vi "ASD Right Sequence Formation.vi"(11 "Sample Sequence":string="TGTXCT") -> (0 "RRS#":i32, 3 "RR Seq":T1)   [LabVIEW 2018]
panel:
  out "逆前削減配列マトリクス":string[][](array[string])
  out "順前削減配列マトリクス":string[][](array[string])
  out "Base#":i32[](array[numeric])
  out "Direction":enum16{"5’→3'", "3'→5'"}[](array[ring])
  out "サイズ":i32
  out "Sequence":string[](array[string])
  out "出力クラスタ":T1
  out "付加配列":string[](array[string])
  out "5' to 3'":string[](array[string])
  out "3' to 5'":string[](array[string])
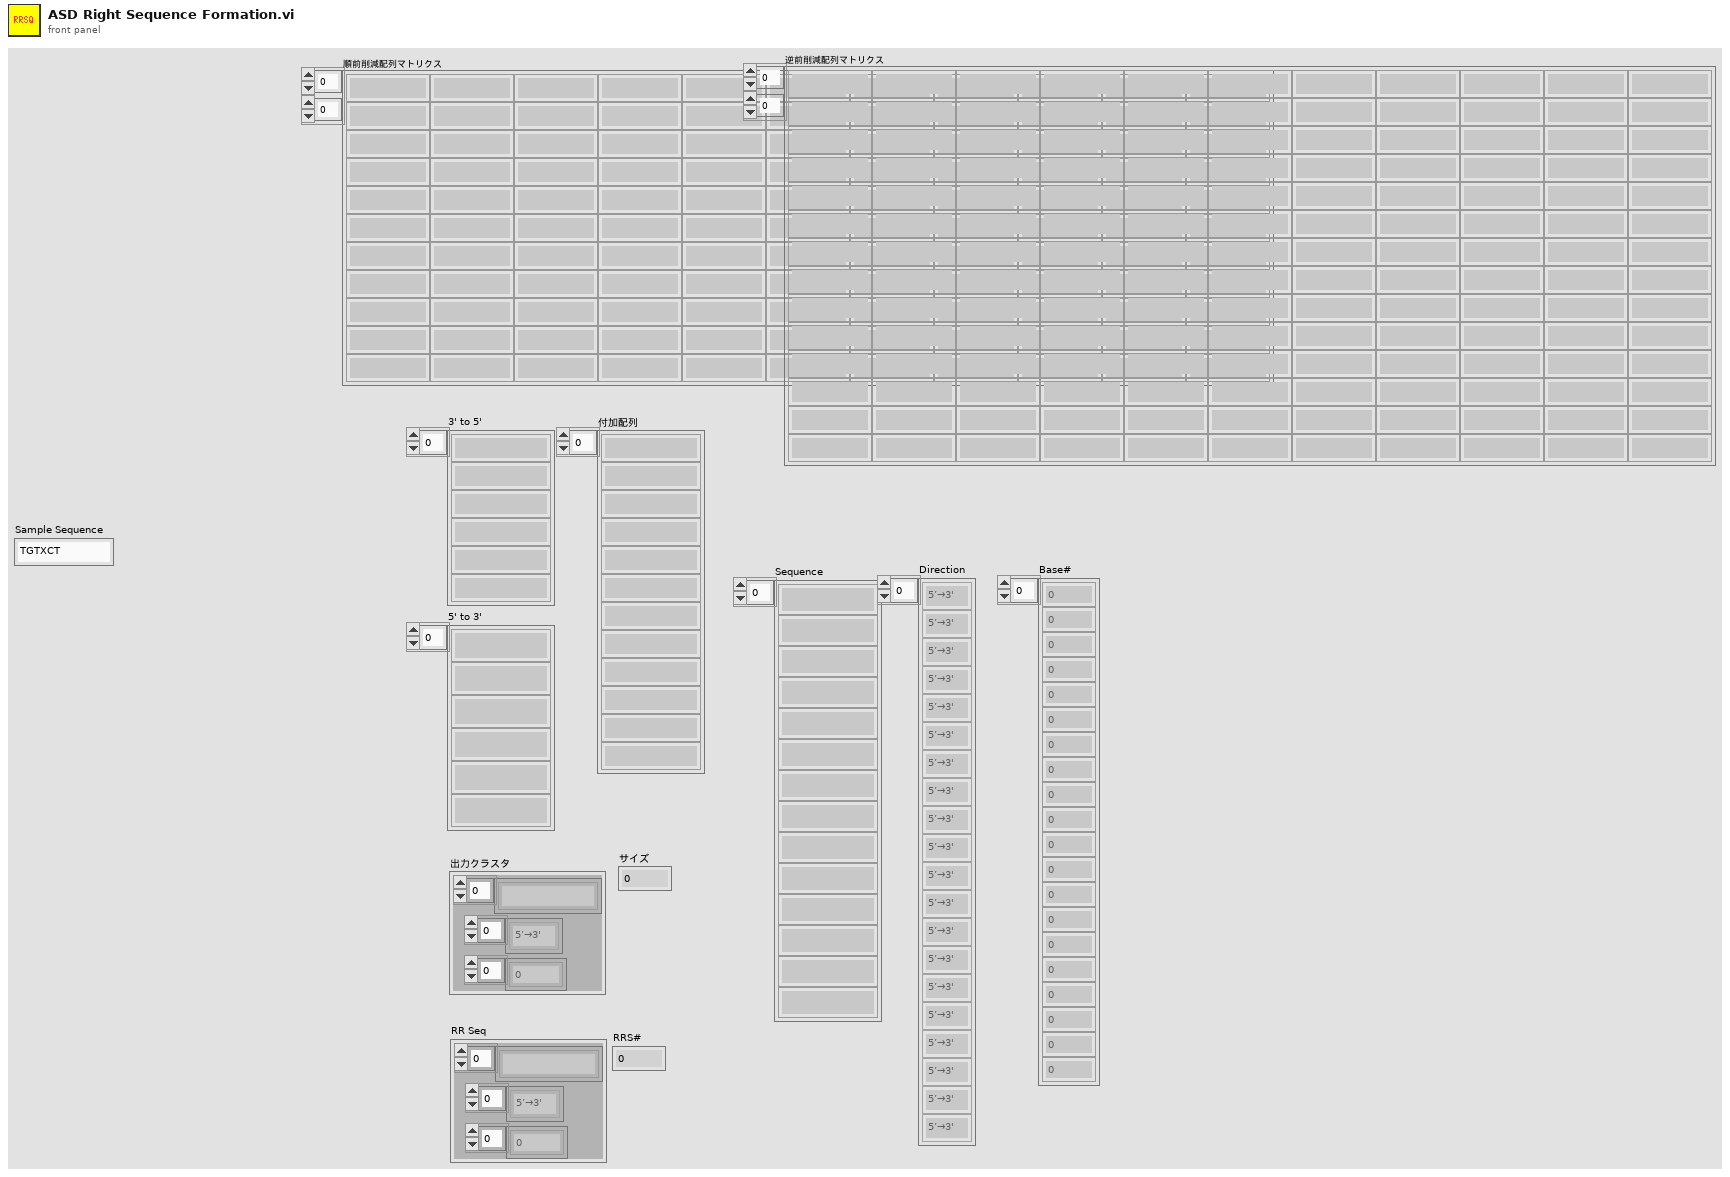
[diagram p1: front panel]
types:
  T1 = cluster{string[], enum16{"5’→3'", "3'→5'"}[], i32[]}
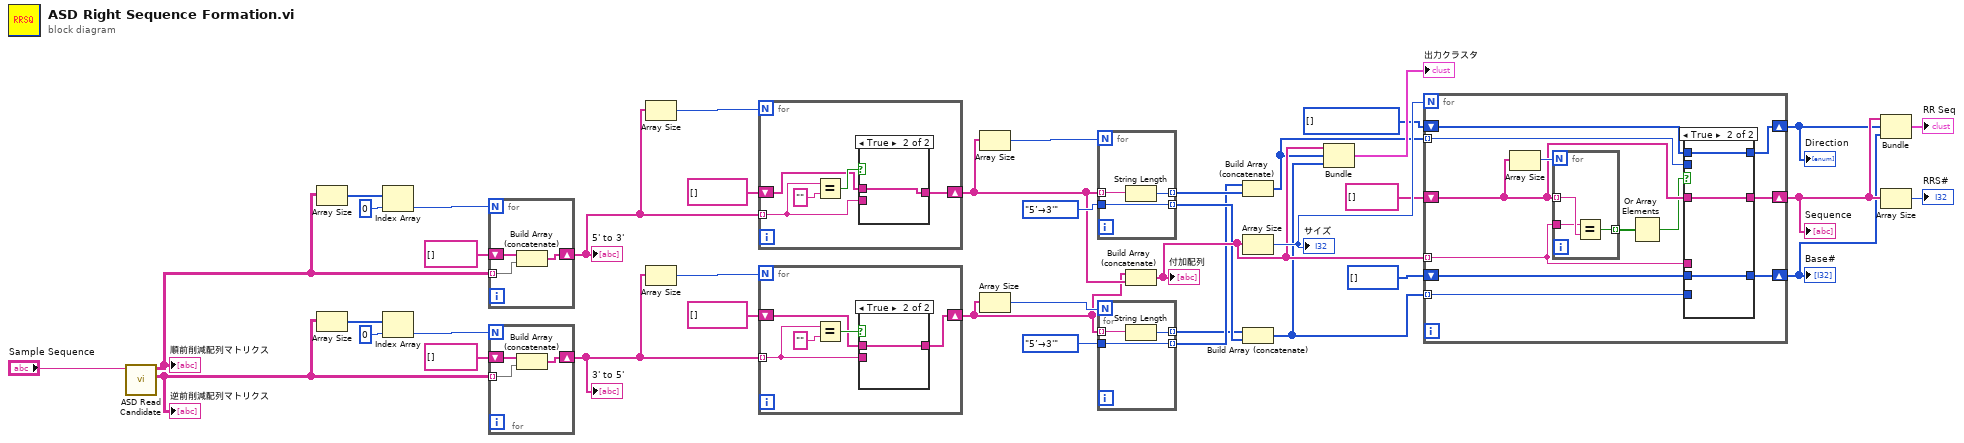
[diagram p0: block diagram]
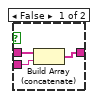
[diagram p2: hidden frame]
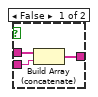
[diagram p3: hidden frame]
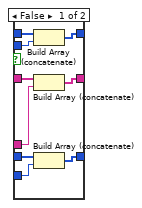
[diagram p4: hidden frame]
diagram:
  w33 = enum16{"5’→3'", "3'→5'"}[] [] items=["5’→3'", "3'→5'"]
  n1 = call "ASD Read Candidate.vi"("読み取り配列"="Sample Sequence") -> ("逆前削減配列マトリクス"=w15:string[][], "順前削減配列マトリクス"=w24:string[][])  [unwired: 8 in, 1 out]
  "順前削減配列マトリクス" <- w24
  "逆前削減配列マトリクス" <- w15
  n2 = Array Size(array=w24) -> (size(s)=w26:i32[])
  n3 = Array Size(array=w15) -> (size(s)=w19:i32[])
  n4 = Index Array(array=w26, index=0 ("指標")) -> (element=w23:i32)
  n5 = Index Array(array=w19, index=0 ("指標")) -> (element=w17:i32)
  n6 = for {
    N: w23 -> [_]
    tunnel: w24 -> [w43] mode=indexing
    shift-right: [w41] -> w4
    shift-left: string[] [] -> [w42]
    n7 = Build Array (concatenate)(w42, w43) -> (w41:string[])
  }
  "5' to 3'" <- w4
  n8 = for {
    N: w17 -> [_]
    tunnel: w15 -> [w46] mode=indexing
    shift-right: [w44] -> w2
    shift-left: string[] [] -> [w45]
    n9 = Build Array (concatenate)(w45, w46) -> (w44:string[])
  }
  "3' to 5'" <- w2
  n10 = Array Size(array=w4) -> (size(s)=w8:i32)
  n11 = Array Size(array=w2) -> (size(s)=w6:i32)
  n12 = for {
    N: w8 -> [_]
    tunnel: w4 -> [w47] mode=indexing
    shift-right: [w48] -> w3
    shift-left: string[] [] -> [w49]
    n13 = Equal?(x=w47, y="") -> (x = y?=w50:bool)
    n14 = case shown="True" w50 {
      tunnel: w49 -> [w54 w55]
      tunnel: [w53 w55] -> w48
      tunnel: w47 -> [w52 _]
      frame False {
        n15 = Build Array (concatenate)(w54, w52) -> (w53:string[])
      }
      frame True {
      }
    }
  }
  n16 = for {
    N: w6 -> [_]
    tunnel: w2 -> [w56] mode=indexing
    shift-right: [w57] -> w1
    shift-left: string[] [] -> [w58]
    n17 = Equal?(x=w56, y="") -> (x = y?=w59:bool)
    n18 = case shown="True" w59 {
      tunnel: w58 -> [w63 w64]
      tunnel: [w62 w64] -> w57
      tunnel: w56 -> [w61 _]
      frame False {
        n19 = Build Array (concatenate)(w63, w61) -> (w62:string[])
      }
      frame True {
      }
    }
  }
  n20 = Array Size(array=w3) -> (size(s)=w21:i32)
  n21 = Array Size(array=w1) -> (size(s)=w14:i32)
  n22 = for {
    N: w21 -> [_]
    tunnel: enum16{"5’→3'", "3'→5'"}."5’→3'" ("リード方向総合") -> [w67]
    tunnel: [w67] -> w12 mode=indexing
    tunnel: w3 -> [w66] mode=indexing
    tunnel: [w65] -> w11 mode=indexing
    n23 = String Length(string=w66) -> (length=w65:i32)
  }
  n24 = for {
    N: w14 -> [_]
    tunnel: enum16{"5’→3'", "3'→5'"}."5’→3'" ("リード方向総合") -> [w70]
    tunnel: [w70] -> w10 mode=indexing
    tunnel: w1 -> [w69] mode=indexing
    tunnel: [w68] -> w9 mode=indexing
    n25 = String Length(string=w69) -> (length=w68:i32)
  }
  n26 = Build Array (concatenate)(w1, w3) -> (w38:string[])
  "付加配列" <- w38
  n27 = Build Array (concatenate)(w10, w11) -> (w34:i32[])
  n28 = Array Size(array=w38) -> (size(s)=w40:i32)
  "サイズ" <- w40
  n29 = Build Array (concatenate)(w9, w12) -> (w35:i32[])
  n30 = Bundle(w38, w34, w35) -> (→"出力クラスタ":cluster{string[], i32[], i32[]})  [unwired: 1 in]
  n31 = for {
    N: w40 -> [_]
    tunnel: w38 -> [w79] mode=indexing
    shift-right: [w82] -> w31
    shift-left: string[] [] -> [w80]
    tunnel: w35 -> [w73] mode=indexing
    tunnel: w34 -> [w76] mode=indexing
    shift-right: [w75] -> w30
    shift-left: w33 -> [w74]
    shift-right: [w72] -> w29
    shift-left: i32[] [] -> [w71]
    n32 = Array Size(array=w80) -> (size(s)=w81:i32)
    n33 = for {
      N: w81 -> [_]
      tunnel: w80 -> [w97] mode=indexing
      tunnel: w79 -> [w96]
      tunnel: [w95] -> w78 mode=indexing
      n34 = Equal?(x=w96, y=w97) -> (x = y?=w95:bool)
    }
    n35 = Or Array Elements(Boolean array=w78) -> (logical OR=w77:bool)
    n36 = case shown="True" w77 {
      tunnel: [w91 w94] -> w82
      tunnel: w80 -> [w90 w94]
      tunnel: w79 -> [w89 _]
      tunnel: w76 -> [w88 _]
      tunnel: [w87 w93] -> w75
      tunnel: w74 -> [w86 w93]
      tunnel: w73 -> [w85 _]
      tunnel: [w84 w92] -> w72
      tunnel: w71 -> [w83 w92]
      frame False {
        n37 = Build Array (concatenate)(w86, w88) -> (w87:i32[])
        n38 = Build Array (concatenate)(w90, w89) -> (w91:string[])
        n39 = Build Array (concatenate)(w83, w85) -> (w84:i32[])
      }
      frame True {
      }
    }
  }
  "Sequence" <- w31
  "Direction" <- w30
  "Base#" <- w29
  n40 = Bundle(w31, w30, w29) -> (→"RR Seq":cluster{string[], i32[], i32[]})  [unwired: 1 in]
  n41 = Array Size(array=w31) -> (size(s)=→"RRS#":i32)
